vi "FinalizeListGeneration.vi"(8 "error in (no error)":errorcluster, 9 "Root path":path, 10 "CDependencyList in":refnum<class "CDependencyList.lvclass">, 11 "CReporter in":refnum<class "CReporter.lvclass">) -> (0 "error out":errorcluster, 3 "CReporter out":refnum<class "CReporter.lvclass">)   [LabVIEW 2020, in "DependencyInspection.lvlib" / "CReporter.lvclass"]
uses:
  CReporter.lvclass
  CDependencyList/CDependencyList.lvclass
  CReporter.lvclass/CReporter.ctl
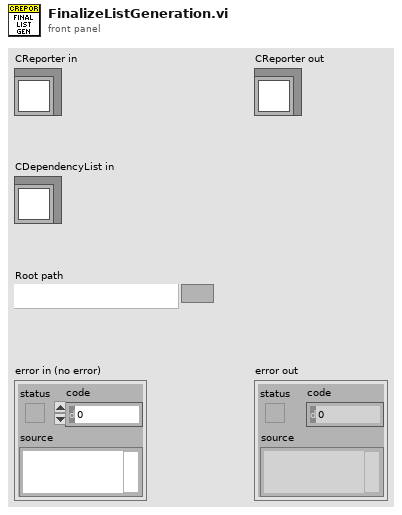
[diagram p1: front panel]
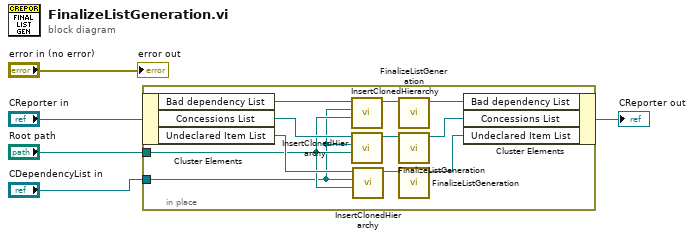
[diagram p0: block diagram]
diagram:
  n1 = in-place {
    in-place-border: "Root path" -> [w13]
    in-place-border: "CDependencyList in" -> [w12]
    n2 = in-place-cluster #1("CReporter in") -> ("Bad dependency List"=w16:refnum<class "CDependencyList.lvclass">, "Concessions List"=w15:refnum<class "CDependencyList.lvclass">, "Undeclared Item List"=w14:refnum<class "CDependencyList.lvclass">)
    n3 = call-dynamic "InsertClonedHierarchy.vi"("Root path"=w13, "Dependency List in"=w12, "CDependencyList in"=w16) -> ("CDependencyList out"=w11:refnum<class "CDependencyList.lvclass">)  [unwired: 7 in, 1 out]
    n4 = call-dynamic "InsertClonedHierarchy.vi"("Root path"=w13, "Dependency List in"=w12, "CDependencyList in"=w15) -> ("CDependencyList out"=w10:refnum<class "CDependencyList.lvclass">)  [unwired: 7 in, 1 out]
    n5 = call-dynamic "InsertClonedHierarchy.vi"("Root path"=w13, "Dependency List in"=w12, "CDependencyList in"=w14) -> ("CDependencyList out"=w9:refnum<class "CDependencyList.lvclass">)  [unwired: 7 in, 1 out]
    n6 = call-dynamic "FinalizeListGeneration.vi"("CDependencyList in"=w11) -> ("CDependencyList out"=w6:refnum<class "CDependencyList.lvclass">)  [unwired: 9 in, 1 out]
    n7 = call-dynamic "FinalizeListGeneration.vi"("CDependencyList in"=w10) -> ("CDependencyList out"=w7:refnum<class "CDependencyList.lvclass">)  [unwired: 9 in, 1 out]
    n8 = call-dynamic "FinalizeListGeneration.vi"("CDependencyList in"=w9) -> ("CDependencyList out"=w8:refnum<class "CDependencyList.lvclass">)  [unwired: 9 in, 1 out]
    n9 = in-place-cluster #1("Bad dependency List"=w6, "Concessions List"=w7, "Undeclared Item List"=w8) -> (→"CReporter out":refnum<class "CReporter.lvclass">)
  }
  "error out" <- "error in (no error)"
